vi "PicoScope3000aSetEtsTimeBuffer.vi"(8 "error in (no error)":errorcluster, 10 "bufferLth":i32, 11 "handle in":i16) -> (0 "error out":errorcluster, 2 "EtsTimeValues":i64[](array[numeric]), 3 "handle out":i16)   [LabVIEW 2010]
doc: "Calls SetEtsTimeBuffer"
uses:
  ps3000a.dll
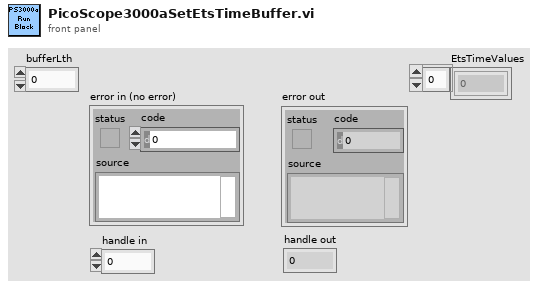
[diagram p1: front panel]
types:
  T1 = enum16{"U8", "I8", "U16", "I16", "U32", "I32", "U64", "I64"}
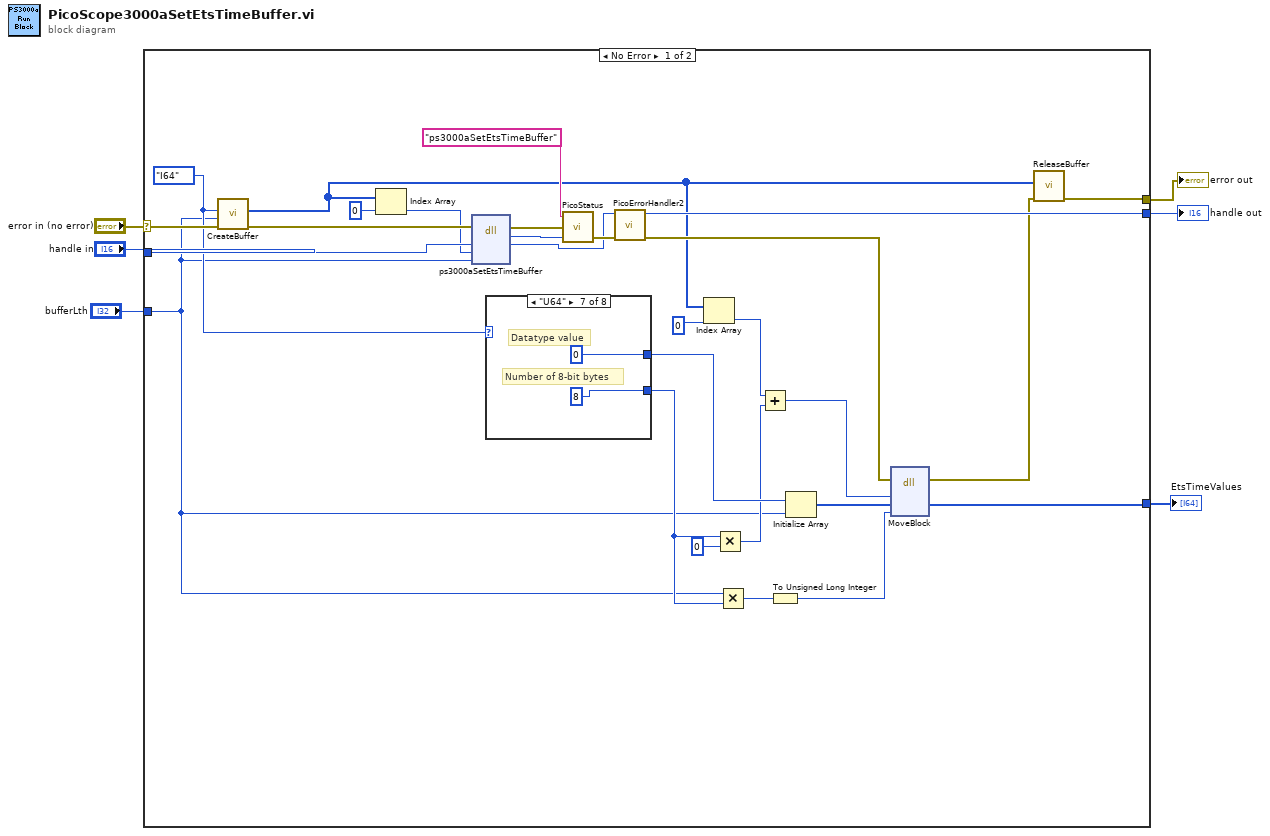
[diagram p0: block diagram]
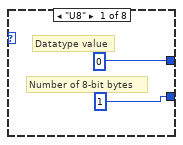
[diagram p2: hidden frame]
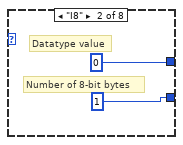
[diagram p3: hidden frame]
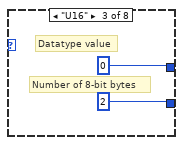
[diagram p4: hidden frame]
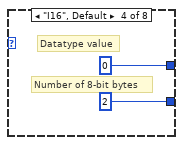
[diagram p5: hidden frame]
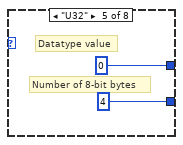
[diagram p6: hidden frame]
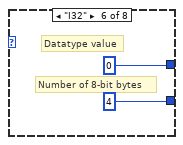
[diagram p7: hidden frame]
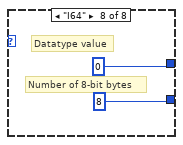
[diagram p8: hidden frame]
diagram:
  n1 = case shown="No Error" "error in (no error)" {
    selector: "error in (no error)" -> [w27 w51]
    tunnel: [w25 w51] -> w4
    tunnel: "handle in" -> [w31 w50]
    tunnel: [w28 w50] -> w5
    tunnel: "bufferLth" -> [w9 _]
    tunnel: [w11 _] -> w1
    frame No Error {
      w14 = T1."I64" ("Data type")
      n2 = call "CreateBuffer.vi"("error in (no error)"=w27, "Buffer size"=w9, "Data type"=w14) -> ("error out"=w26:errorcluster, "Pointer and BufferSize"=w8:u64[])  [unwired: 7 in]
      n3 = Index Array(array=w8, index=0) -> (element=w24:u64)
      n4 = dll-call lib="ps3000a.dll" fn="ps3000aSetEtsTimeBuffer" ("ps3000.dll:_ps3000_open_unit@0")(error in=w26, "handle"=w31, "buffer"=w24, "bufferLth"=w9) -> (error out=w30:errorcluster, "PICO_STATUS"=w29:u32, "handle"=w28:i16)  [unwired: 4 in, 1 out]
      n5 = case shown="\"U64\"" w14 {
        tunnel: [u8 0 ("element") i8 0 ("element") u16 0 ("element") i16 0 ("element") u32 0 ("element") 0 ("element") u64 0 ("element") i64 0 ("element")] -> w22
        tunnel: [u64 1 ("y") u64 1 ("y") u64 2 ("y") u64 2 ("y") u64 4 ("y") u64 4 ("y") u64 8 ("y") u64 8 ("y")] -> w19
        frame "U8" {
          # "Number of 8-bit bytes"
          # "Datatype value"
        }
        frame "I8" {
          # "Number of 8-bit bytes"
          # "Datatype value"
        }
        frame "U16" {
          # "Number of 8-bit bytes"
          # "Datatype value"
        }
        frame "I16", Default {
          # "Number of 8-bit bytes"
          # "Datatype value"
        }
        frame "U32" {
          # "Number of 8-bit bytes"
          # "Datatype value"
        }
        frame "I32" {
          # "Number of 8-bit bytes"
          # "Datatype value"
        }
        frame "U64" {
          # "Number of 8-bit bytes"
          # "Datatype value"
        }
        frame "I64" {
          # "Number of 8-bit bytes"
          # "Datatype value"
        }
      }
      n6 = call "PicoStatus.vi"("PICO STATUS"=w29, "error in"=w30, "source"="ps3000aSetEtsTimeBuffer") -> ("error out"=w33:errorcluster)
      n7 = call "PicoErrorHandler2.vi"("error in (no error)"=w33, "handle In"=w28) -> ("error out"=w12:errorcluster)  [unwired: 9 in]
      n8 = Index Array(array=w8, index=0) -> (element=w21:u64)
      n9 = Multiply(x=w19, y=u64 0) -> (x*y=w20:u64)
      n10 = Multiply(x=w9, y=w19) -> (x*y=w18:u64)
      n11 = Add(x=w21, y=w20) -> (x+y=w17:u64)
      n12 = To Unsigned Long Integer(number=w18) -> (unsigned 32bit integer=w15:u32)
      n13 = Initialize Array(w22, w9) -> (w16:u64[])
      n14 = dll-call lib="LabVIEW" fn="MoveBlock"(error in=w12, "Source"=w17, "Destination"=w16, "Size"=w15) -> (error out=w13:errorcluster, "Destination"=w11:i64[])  [unwired: 5 in, 1 out]
      n15 = call "ReleaseBuffer.vi"("error in (no error)"=w13, "Pointer and BufferSize"=w8) -> ("error out"=w25:errorcluster)  [unwired: 9 in]
    }
    frame Error {
    }
  }
  "error out" <- w4
  "handle out" <- w5
  "EtsTimeValues" <- w1
